vi "Test_C_Codec_RoundTrip.vi"() -> ()   [LabVIEW 2021]
uses:
  CANsub_C.lvlib
panel:
  out "checked":i32
  out "mismatches":u32
  out "error out":errorcluster
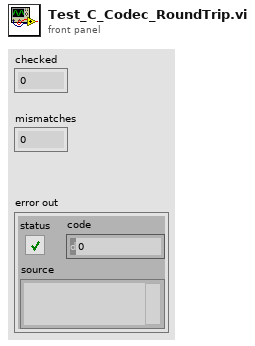
[diagram p1: front panel]
types:
  T1 = typedef "CANsub_C.lvlib/C_State.ctl" = u8[]
  T2 = typedef "CANsub_Common.lvlib/Payload.ctl" = cluster{"payload":T3}
  T3 = typedef "CANsub_Common.lvlib/Bytes.ctl" = u8[]
  T4 = typedef "CANsub_Common.lvlib/CAN_Frame.ctl" = cluster{"t_dev":dbl, "id":u32, "ide":bool, "fdf":bool, "rtr":bool, "brs":bool, "esi":bool, "tx_ack":bool, "error":bool, "err type":u8, "dlc":u8, "data":T3}
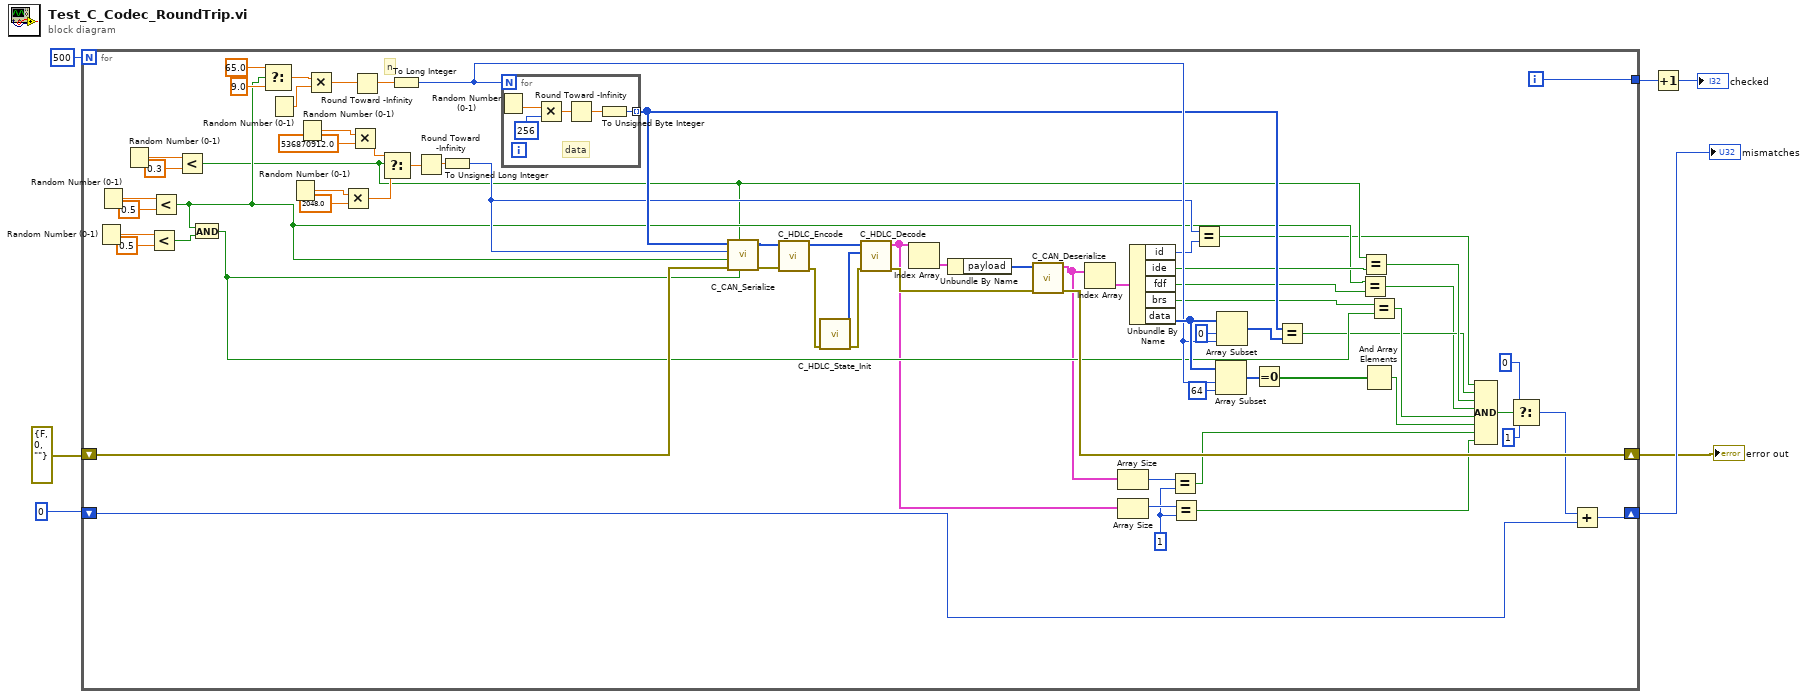
[diagram p0: block diagram]
diagram:
  n1 = for {
    N: 500 -> [_]
    shift-right: [w18] -> w4
    shift-left: u32 0 -> [w20]
    shift-right: [w45] -> w3
    shift-left: errorcluster {"status"=FALSE, "code"=0, "source"=""} ("error out") -> [w50]
    tunnel: [w8] -> w2
    i -> [w8]
    w25 = 1
    # "n"
    n2 = Random Number (0-1)() -> (number: 0 to 1=w73:dbl)
    n3 = Random Number (0-1)() -> (number: 0 to 1=w76:dbl)
    n4 = Random Number (0-1)() -> (number: 0 to 1=w70:dbl)
    n5 = Less?(x=w73, y=0.5) -> (x < y?=w72:bool)
    n6 = Less?(x=w76, y=0.5) -> (x < y?=w30:bool)
    n7 = Less?(x=w70, y=0.3) -> (x < y?=w29:bool)
    n8 = And(x=w30, y=w72) -> (x .and. y?=w31:bool)
    n9 = Select(t=65.0, s=w30, f=9.0) -> (s? t:f=w59:dbl)
    n10 = Random Number (0-1)() -> (number: 0 to 1=w58:dbl)
    n11 = Random Number (0-1)() -> (number: 0 to 1=w66:dbl)
    n12 = Random Number (0-1)() -> (number: 0 to 1=w69:dbl)
    n13 = Multiply(x=w59, y=w58) -> (x*y=w57:dbl)
    n14 = Multiply(x=w66, y=2048.0) -> (x*y=w64:dbl)
    n15 = Multiply(x=w69, y=536870912.0) -> (x*y=w65:dbl)
    n16 = Round Toward -Infinity(1:w57) -> (0:w56:dbl)
    n17 = Select(t=w65, s=w29, f=w64) -> (s? t:f=w63:dbl)
    n18 = To Long Integer(number=w56) -> (32bit integer=w43:i32)
    n19 = Round Toward -Infinity(1:w63) -> (0:w62:dbl)
    n20 = To Unsigned Long Integer(number=w62) -> (unsigned 32bit integer=w35:u32)
    n21 = for {
      N: w43 -> [_]
      tunnel: [w77] -> w37 mode=indexing
      # "data"
      n22 = Random Number (0-1)() -> (number: 0 to 1=w81:dbl)
      n23 = Multiply(x=w81, y=256) -> (x*y=w79:dbl)
      n24 = Round Toward -Infinity(1:w79) -> (0:w78:dbl)
      n25 = To Unsigned Byte Integer(number=w78) -> (unsigned 8bit integer=w77:u8)
    }
    n26 = call "C_CAN_Serialize.vi"("brs"=w31, "ide"=w29, "error in (no error)"=w50, "fdf"=w30, "id"=w35, "data"=w37) -> ("error out"=w49:errorcluster, "payload"=w55:u8[])  [unwired: 4 in]
    n27 = call "C_HDLC_Encode.vi"("error in (no error)"=w49, "payload"=w55) -> ("error out"=w48:errorcluster, "frame"=w54:u8[])  [unwired: 8 in]
    n28 = call "C_HDLC_State_Init.vi"("error in (no error)"=w48) -> ("error out"=w47:errorcluster, "C_State"=w53:T1)  [unwired: 9 in]
    n29 = call "C_HDLC_Decode.vi"("error in (no error)"=w47, "state in"=w53, "bytes in"=w54) -> ("error out"=w46:errorcluster, "payloads"=w9:T2[])  [unwired: 5 in, 2 out]
    n30 = Index Array(array=w9) -> (element=w52:T2)  [unwired: 1 in]
    n31 = Unbundle By Name(w52) -> ("payload"=w28:T3)
    n32 = call "C_CAN_Deserialize.vi"("error in (no error)"=w46, "payload"=w28) -> ("error out"=w45:errorcluster, "frames"=w27:T4[])  [unwired: 7 in, 1 out]
    n33 = Index Array(array=w27) -> (element=w51:T4)  [unwired: 1 in]
    n34 = Array Size(array=w27) -> (size(s)=w24:i32)
    n35 = Array Size(array=w9) -> (size(s)=w26:i32)
    n36 = Unbundle By Name(w51) -> ("id"=w36:u32, "ide"=w34:bool, "fdf"=w33:bool, "brs"=w32:bool, "data"=w44:T3)
    n37 = Equal?(x=w24, y=w25) -> (x = y?=w12:bool)
    n38 = Equal?(x=w26, y=w25) -> (x = y?=w11:bool)
    n39 = Equal?(x=w35, y=w36) -> (x = y?=w17:bool)
    n40 = Array Subset(array=w44, index=w43, length=64) -> (w40:T3)
    n41 = Array Subset(array=w44, index=0, length=w43) -> (w38:T3)
    n42 = Equal To 0?(x=w40) -> (x = 0?=w39:bool[])
    n43 = Equal?(x=w37, y=w38) -> (x = y?=w14:bool)
    n44 = Equal?(x=w30, y=w33) -> (x = y?=w10:bool)
    n45 = Equal?(x=w29, y=w34) -> (x = y?=w16:bool)
    n46 = And Array Elements(Boolean array=w39) -> (logical AND=w13:bool)
    n47 = Equal?(x=w32, y=w31) -> (x = y?=w15:bool)
    n48 = Compound Arithmetic op=AND(w17, w14, w16, w10, w15, w13, w12, w11) -> (w23:bool)
    n49 = Select(t=0, s=w23, f=1) -> (s? t:f=w19:i32)
    n50 = Add(x=w19, y=w20) -> (x+y=w18:u32)
  }
  "error out" <- w3
  "mismatches" <- w4
  n51 = Increment(x=w2) -> (x+1=→"checked":i32)
